vi "Tile_Read.vi"(0 "Tiles":u8[][](array[numeric]), 5 "X":i32, 7 "Y":i32, 11 "error in":errorcluster) -> (4 "Tile":u8, 15 "error out":errorcluster)   [LabVIEW 2020, in "GH_Level.lvlib"]
doc: "Tile value under the point (X, Y) in playfield pixels (tile = 32 px). Points outside the room read the nearest tile at the edge, so a ladder, pole or floor that leaves the room continues until the room changes."
uses:
  GH_Level.lvlib
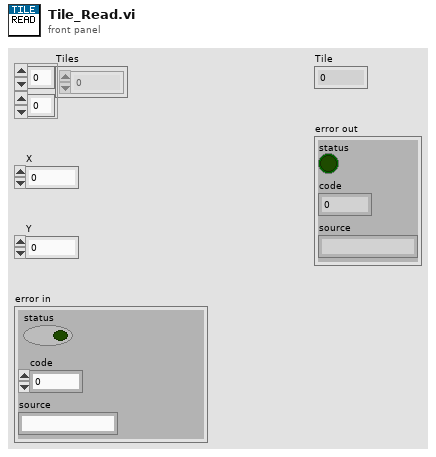
[diagram p1: front panel]
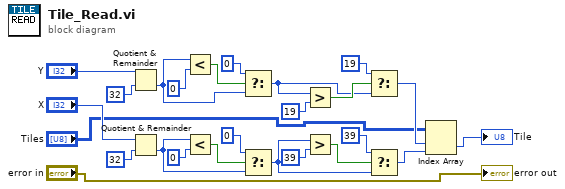
[diagram p0: block diagram]
diagram:
  n1 = Quotient & Remainder(x="Y", y=32) -> (floor(x/y)=w8:i32)  [unwired: 1 out]
  n2 = Quotient & Remainder(x="X", y=32) -> (floor(x/y)=w6:i32)  [unwired: 1 out]
  n3 = Less?(x=w8, y=0) -> (x < y?=w10:bool)
  n4 = Less?(x=w6, y=0) -> (x < y?=w18:bool)
  n5 = Select(t=0, s=w10, f=w8) -> (s? t:f=w12:i32)
  n6 = Select(t=0, s=w18, f=w6) -> (s? t:f=w20:i32)
  n7 = Greater?(x=w12, y=19) -> (0:w14:bool)
  n8 = Greater?(x=w20, y=39) -> (0:w22:bool)
  n9 = Select(t=19, s=w14, f=w12) -> (s? t:f=w16:i32)
  n10 = Select(t=39, s=w22, f=w20) -> (s? t:f=w24:i32)
  n11 = Index Array(array="Tiles", index (row)=w16, index (col)=w24) -> (element=→"Tile":u8)
  "error out" <- "error in"
